vi "RT_Protective_Response.vi"(8 "error in (no error)":errorcluster={"status"=FALSE, "code"=0, "source"="\"\""}, 10 "rig safety policy":string, 11 "Latched fault type":string) -> (0 "error out":errorcluster={"status"=FALSE, "code"=0, "source"="\"\""}, 2 "status ok":bool, 3 "Protective action result":string)   [LabVIEW 2026]
doc: "INTENT: Request approved safe control behavior. LOGIC: Invoke approved actuator disable/vent/hold strategy only if available and safe; report fallback status."
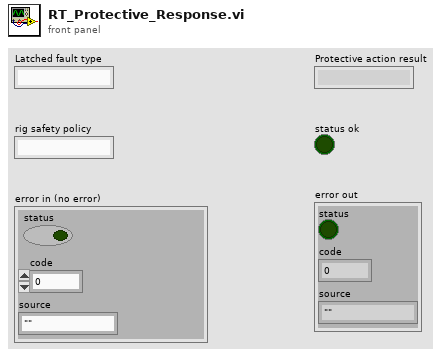
[diagram p1: front panel]
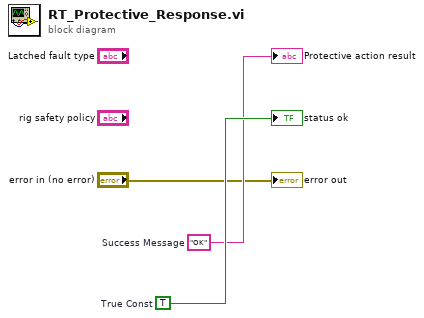
[diagram p0: block diagram]
diagram:
  w3 = TRUE  # True Const
  w2 = "OK"  # Success Message
  "Protective action result" <- w2
  "status ok" <- w3
  "error out" <- "error in (no error)"
